vi "WPI_RobotDriveMecanumDrive_Polar.vi"(6 "Rotation":dbl, 8 "error in (no error)":errorcluster, 9 "Direction":dbl, 10 "Magnitude":dbl, 11 "RobotDriveDevRef":T1={"Motors[]"=[], "Square Inputs"=FALSE, "Max Output"=1.0}) -> (0 "error out":errorcluster, 2 "Motor Values":dbl[](array[numeric]), 3 "RobotDriveDevRef":T1={"Motors[]"=[], "Square Inputs"=FALSE, "Max Output"=1.0})   [LabVIEW 2023]
doc: "Configures the motors for holonomic driving. Holonomic driving allows you to move the robot in any direction without first rotating or maneuvering the robot.\n\nThis VI requires the robot to have either four omni-directional wheels and four motors mounted at 45 degree angles in the four corners of a square frame or to have four mecanum wheels driven by four motors.\n\nThe control input is intended to come from autonomous code or any other time that polar notation is convenient.\n\nThis software is licensed. Open the labview\\readme\\WPI Robotics Library Open Source License.txt file for more information."
uses:
  <vilib>/Rock Robotics/WPI/RobotDrive/WPI_RobotDriveDevRef.ctl
  <vilib>/REV Custom Controls/REVSparkRefnum.ctl
  <vilib>/REVLibDriver/REVLibDriver.lvlib
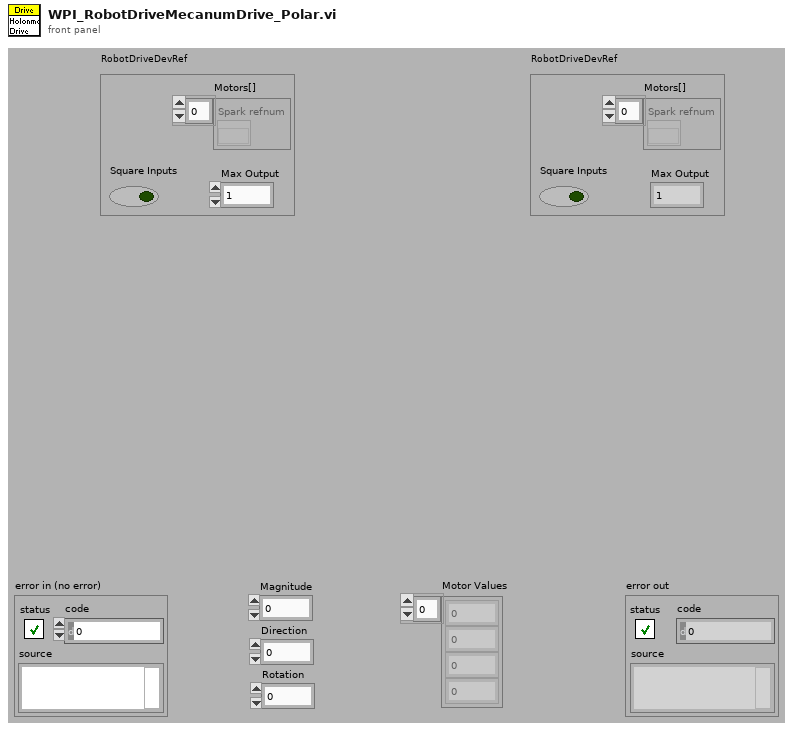
[diagram p1: front panel]
types:
  T1 = typedef "WPI_RobotDriveDevRef.ctl" = cluster{"Motors[]":T2[], "Square Inputs":bool, "Max Output":dbl}
  T2 = typedef "REVLibDriver.lvlib/REVSparkRefnum.ctl" = refnum<k20>
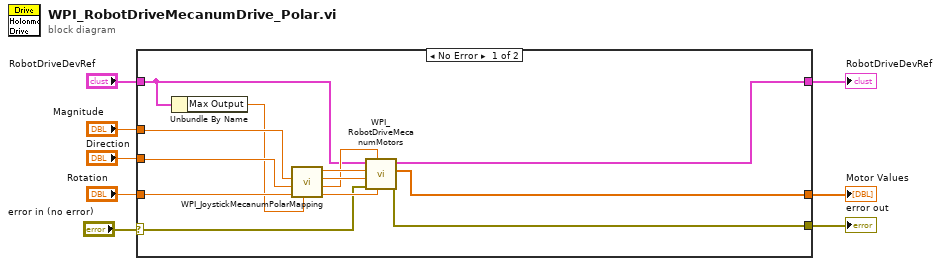
[diagram p0: block diagram]
diagram:
  n1 = case shown="No Error" "error in (no error)" {
    selector: "error in (no error)" -> [w11 w23]
    tunnel: "Direction" -> [w17 _]
    tunnel: "Magnitude" -> [w16 _]
    tunnel: "RobotDriveDevRef" -> [w10 w22]
    tunnel: [w19 w22] -> w4
    tunnel: [w20 w23] -> w3
    tunnel: "Rotation" -> [w18 _]
    tunnel: [w21 _] -> w1
    frame No Error {
      n2 = Unbundle By Name(w10) -> ("Max Output"=w9:dbl)
      n3 = call <vilib>:"WPI_JoystickMecanumPolarMapping.vi"("Max Output"=w9, "Rotation"=w18, "Direction"=w17, "Magnitude"=w16) -> ("Rear Right"=w12:dbl, "Rear Left"=w13:dbl, "Front Right"=w14:dbl, "Front Left"=w15:dbl)  [unwired: 4 in]
      n4 = call <vilib>:"WPI_RobotDriveMecanumMotors.vi"("Rear Right"=w12, "Rear Left"=w13, "error in"=w11, "Front Right"=w14, "Front Left"=w15, "RobotDriveDevRef in"=w10) -> ("error out"=w20:errorcluster, "Motor Values"=w21:dbl[], "RobotDriveDevRef out"=w19:T1)  [unwired: 3 in]
    }
    frame Error {
    }
  }
  "error out" <- w3
  "RobotDriveDevRef" <- w4
  "Motor Values" <- w1
